vi "_Publish DP Indicators(Refmgr).vi"(7 "VIRef(Caller VI)":refnum<k1>, 8 "error in (no error)":errorcluster, 9 "force update(F)":bool, 11 "SILAPI In":refnum<k1>) -> (0 "error out":errorcluster, 1 "Binded DPs":string[](array[string]), 3 "SILAPI Out":refnum<k1>)   [LabVIEW 2017, in "TagDB RefManager.lvlib"]
uses:
  TagDB RefManager.lvlib
  10d0bc68-ff5b-4b3e-94b6-72122e87f5c0.vi
  99199be5-3273-4500-92d5-279e96ad7927.vi
  9ac63a17-9284-407c-a5c8-8910fcebbfe1.vi
  0f9c47dc-4cad-44a4-9ff9-6b222f0d776a.vi
  <userlib>/_NEVSTOP/TagDB/_Support/DataAccess/_NameCacher.vi
  <userlib>/_NEVSTOP/TagDB/_Support/Error/_[error50002]Invalid DataType.vi
  <userlib>/_NEVSTOP/TagDB/_Support/Error/_[error50000]Invalid DB REF.vi
  <userlib>/_NEVSTOP/TagDB/_Support/DataAccess/TagDB Ref to DVR.vi
  <userlib>/_NEVSTOP/TagDB/_Support/URL/TRIM-BOTH-SPACE.vi
  9ac63a17-9284-407c-a5c8-8910fcebbfe1.vi/1b47866c-8e2d-43a7-815f-8cf18635e5a1.vi
  0f9c47dc-4cad-44a4-9ff9-6b222f0d776a.vi/1b47866c-8e2d-43a7-815f-8cf18635e5a1.vi
  <userlib>/_NEVSTOP/TagDB/_Support/Change Detector/TagDB dbChanged.vi
  <userlib>/_NEVSTOP/TagDB/_Support/Error/_Clear Errors.vi
  9ac63a17-9284-407c-a5c8-8910fcebbfe1.vi/1b47866c-8e2d-43a7-815f-8cf18635e5a1.vi/29b2ea6d-6d7f-4e4a-ad31-a5cb760462c7.vi
  <userlib>/_NEVSTOP/TagDB/API/TagDB-Status.vi
  0f9c47dc-4cad-44a4-9ff9-6b222f0d776a.vi/1b47866c-8e2d-43a7-815f-8cf18635e5a1.vi/29b2ea6d-6d7f-4e4a-ad31-a5cb760462c7.vi
  <userlib>/_NEVSTOP/TagDB/_Support/Error/_Build Error Cluster.vi
  <userlib>/_NEVSTOP/TagDB/TagDB.lvlib
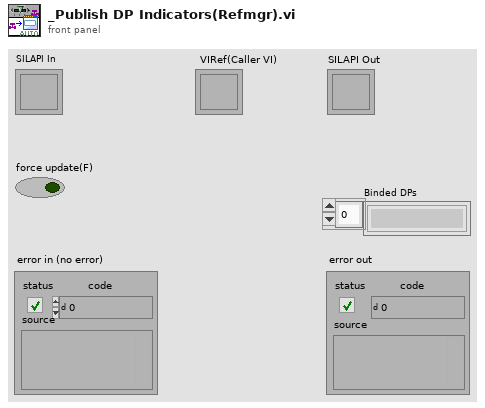
[diagram p1: front panel]
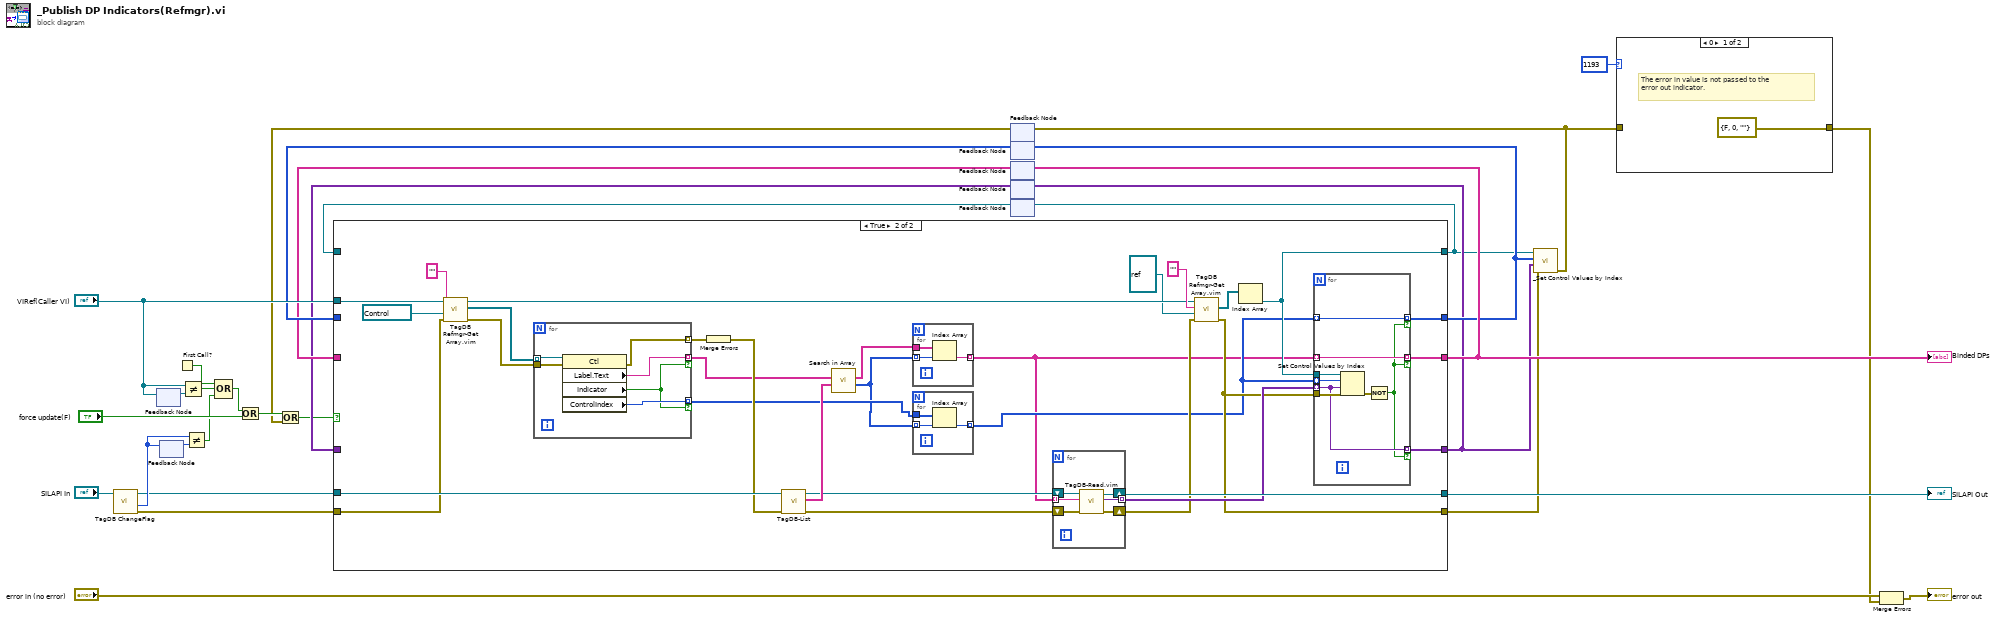
[diagram p0: block diagram]
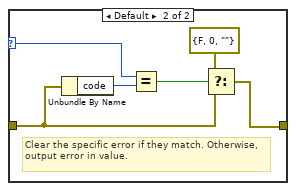
[diagram p2: hidden frame]
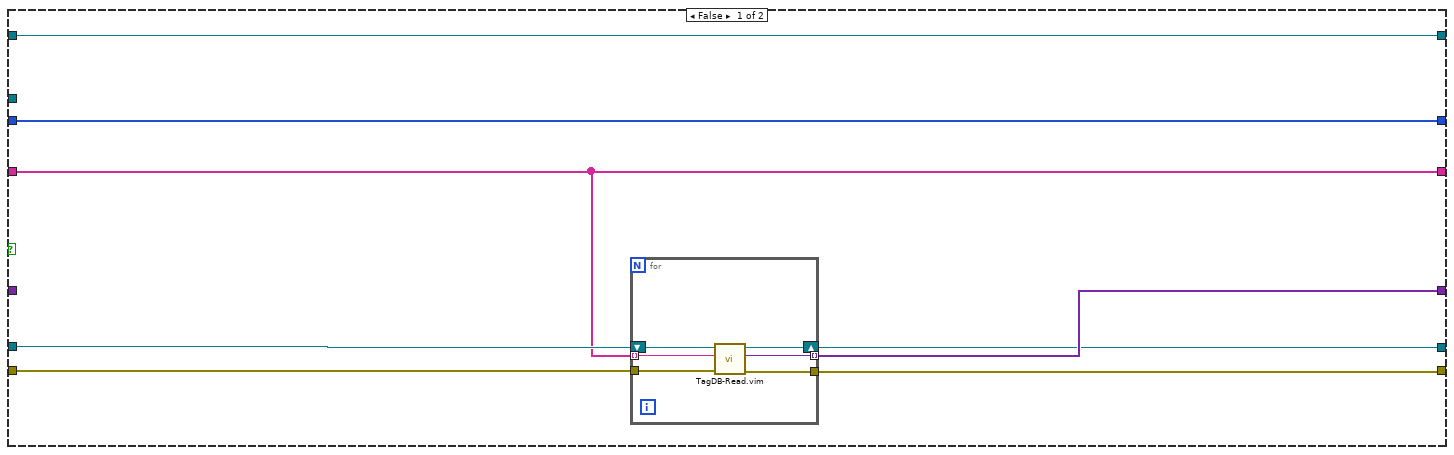
[diagram p3: hidden frame]
diagram:
  n1 = call <userlib>:"TagDB ChangeFlag.vi"("DB Ref"="SILAPI In") -> ("error in (no error) (dup)"=w1:errorcluster, "Item Change Timestamp"=w5:u64, "DB Ref (dup)"=w3:refnum<k1>)  [unwired: 7 in, 1 out]
  n2 = feedback #1() -> (w10:refnum<k1>)  [unwired: 1 in]
  n3 = feedback-in #1("VIRef(Caller VI)") -> ()
  n4 = feedback #2() -> (w6:u64)  [unwired: 1 in]
  n5 = feedback-in #2(w5) -> ()
  n6 = First Call?() -> (First Call?: T/F=w8:bool)
  n7 = Not Equal?(x="VIRef(Caller VI)", y=w10) -> (x != y?=w9:bool)
  n8 = Not Equal?(x=w5, y=w6) -> (x != y?=w2:bool)
  n9 = Compound Arithmetic op=OR(w8, w9, w2) -> (w7:bool)
  n10 = Or(x=w7, y="force update(F)") -> (x .or. y?=w22:bool)
  n11 = feedback #3() -> (w14:errorcluster)  [unwired: 1 in]
  n12 = Or(x=w22, y=w14) -> (x .or. y?=w16:bool)
  n13 = feedback #4() -> (w23:i32[])  [unwired: 1 in]
  n14 = feedback #5() -> (w21:string[])  [unwired: 1 in]
  n15 = feedback #6() -> (w18:variant[])  [unwired: 1 in]
  n16 = feedback #7() -> (w11:refnum<vi>)  [unwired: 1 in]
  n17 = case shown="True" w16 {
    tunnel: [w32 w52] -> w12
    tunnel: "VIRef(Caller VI)" -> [_ w74]
    tunnel: [w38 w68] -> w24
    tunnel: w23 -> [w38 _]
    tunnel: [w36 w69] -> w27
    tunnel: w21 -> [w36 _]
    tunnel: [w34 w67] -> w19
    tunnel: w3 -> [w37 w73]
    tunnel: [w35 w53] -> w20
    tunnel: w18 -> [_ _]
    tunnel: [w33 w71] -> w25
    tunnel: w11 -> [w32 _]
    tunnel: w1 -> [w31 w45]
    frame False {
      n18 = for {
        tunnel: w36 -> [w43] mode=indexing
        tunnel: [w42] -> w35
        tunnel: [w41] -> w34 mode=indexing
        shift-right: [w40] -> w33
        shift-left: w37 -> [w44]
        tunnel: w31 -> [w39]
        n19 = call "TagDB-Read.vim"("error in (no error)"=w39, "name"=w43, "TagDB"=w44) -> ("error out"=w42:errorcluster, "Value"=w41:variant, "TagDB(dup)"=w40:refnum<k1>)  [unwired: 3 in, 3 out]
      }
    }
    frame True {
      n20 = call "TagDB Refmgr-Get Array.vim"("error in (no error)"=w45, "Type"=refnum<vi> refnum, "RegExp"="", "DB Ref"=w74) -> ("error out"=w60:errorcluster, "References"=w59:refnum<vi>[], "DB Ref(dup)"=w57:refnum<k1>)  [unwired: 4 in, 1 out]
      n21 = for {
        tunnel: w59 -> [w92] mode=indexing
        tunnel: [w91] -> w47 mode=indexing if=w89
        tunnel: [w90] -> w50 mode=indexing if=w89
        tunnel: [w88] -> w66 mode=indexing
        tunnel: w60 -> [w87]
        n22 = property class="Ctl"(reference=w92, error in=w87) -> (error out=w88:errorcluster, "Label.Text"=w91:string, "Indicator"=w89:bool, "ControlIndex"=w90:i32)  [unwired: 1 out]
      }
      n23 = Merge Errors(w66) -> (w65:errorcluster)
      n24 = call <userlib>:"TagDB-List.vi"("error in (no error)"=w65, "TagDB"=w73) -> ("error out"=w72:errorcluster, "names"=w64:string[], "TagDB(dup)"=w63:refnum<k1>)  [unwired: 6 in, 1 out]
      n25 = call "Search in Array.vi"("items to filter"=w64, "array"=w47) -> ("item Indexs"=w48:i32[], "array(dup)"=w46:string[])  [unwired: 4 in]
      n26 = for {
        tunnel: w48 -> [w77] mode=indexing
        tunnel: w46 -> [w76]
        tunnel: [w75] -> w49 mode=indexing
        n27 = Index Array(array=w76, index=w77) -> (element=w75:string)
      }
      n28 = for {
        tunnel: w48 -> [w80] mode=indexing
        tunnel: w50 -> [w79]
        tunnel: [w78] -> w51 mode=indexing
        n29 = Index Array(array=w79, index=w80) -> (element=w78:i32)
      }
      n30 = for {
        tunnel: [w84] -> w70 mode=indexing
        tunnel: w49 -> [w82] mode=indexing
        shift-right: [w83] -> w54
        shift-left: w72 -> [w86]
        shift-right: [w85] -> w71
        shift-left: w63 -> [w81]
        n31 = call "TagDB-Read.vim"("error in (no error)"=w86, "name"=w82, "TagDB"=w81) -> ("error out"=w83:errorcluster, "Value"=w84:variant, "TagDB(dup)"=w85:refnum<k1>)  [unwired: 3 in, 3 out]
      }
      n32 = call "TagDB Refmgr-Get Array.vim"("error in (no error)"=w54, "Type"=refnum<vi> refnum ("Current VI Reference"), "RegExp"="", "DB Ref"=w57) -> ("error out"=w53:errorcluster, "References"=w55:refnum<vi>[])  [unwired: 4 in, 2 out]
      n33 = Index Array(array=w55) -> (element=w52:refnum<vi>)  [unwired: 1 in]
      n34 = for {
        tunnel: w52 -> [w100]
        tunnel: w51 -> [w99] mode=indexing
        tunnel: w70 -> [w95] mode=indexing
        tunnel: w53 -> [w98]
        tunnel: [w97] -> w69 mode=indexing if=w93
        tunnel: w49 -> [w97] mode=indexing
        tunnel: [w96] -> w68 mode=indexing if=w93
        tunnel: w51 -> [w96] mode=indexing
        tunnel: [w95] -> w67 mode=indexing if=w93
        n35 = Set Control Values by Index(0:w100, 1:w99, 2:w95, 3:w98) -> (11:w94:errorcluster)
        n36 = Not(x=w94) -> (.not. x?=w93:bool)
      }
    }
  }
  "SILAPI Out" <- w25
  "Binded DPs" <- w27
  n37 = feedback-in #4(w24) -> ()
  n38 = feedback-in #5(w27) -> ()
  n39 = feedback-in #6(w19) -> ()
  n40 = feedback-in #7(w12) -> ()
  n41 = call <userlib>:"_Set Control Values by Index.vi"("error in (no error)"=w20, "data values"=w19, "control indexes"=w24, "VI Refnum"=w12) -> ("error out"=w15:errorcluster)  [unwired: 7 in]
  n42 = feedback-in #3(w15) -> ()
  n43 = case shown="0" 1193 ("specific error code to clear (0: all)") {
    selector: 1193 ("specific error code to clear (0: all)") -> [_ w106]
    tunnel: w15 -> [_ w105]
    tunnel: [errorcluster {"status"=FALSE, "code"=0, "source"=""} ("error constant") w102] -> w17
    frame 0 {
      # "The error in value is not passed to the\nerror out indicator."
    }
    frame Default {
      # "Clear the specific error if they match. Otherwise, output error in value."
      n44 = Unbundle By Name(w105) -> ("code"=w107:i32)
      n45 = Equal?(x=w106, y=w107) -> (x = y?=w103:bool)
      n46 = Select(t=errorcluster {"status"=FALSE, "code"=0, "source"=""} ("error constant"), s=w103, f=w105) -> (s? t:f=w102:errorcluster)
    }
  }
  n47 = Merge Errors("error in (no error)", w17) -> (→"error out":errorcluster)
